vi "ntc_view.vi"() -> ()   [LabVIEW 2026]
uses:
  <vilib>/Instr/_visa.llb/VISA Configure Serial Port (Instr).vi
  <vilib>/express/express shared/transition.llb/Dynamic To Waveform Array.vi
  <vilib>/express/express signal manip/GetorSetDDTAttributes/Set DDT Attributes/SetT0.vi
  <vilib>/express/express shared/transition.llb/Waveform Array To Dynamic.vi
  <vilib>/express/express signal manip/GetorSetDDTAttributes/Set DDT Attributes/Set DDT Properties.xnode
panel:
  out "GOOD":bool
  out "Alarm <=  17 °C":bool
  out "Alarm\n >= 37 °C":bool caption="x >= y?"
  out "Linear Checker":cluster{"Tensão":dbl, "Waveform Chart":dbl}[](graph)
  out "Temperature Vs Time":dbl(graph)
  out "ADC Raw":u32
  out "Tensão":dbl(knob) scale=0.0..10.0
  out "Temperatura":dbl(slide) scale=17.0..37.0
  in  "stop":bool
  in  "VISA resource name":refnum<visa-resource-name>
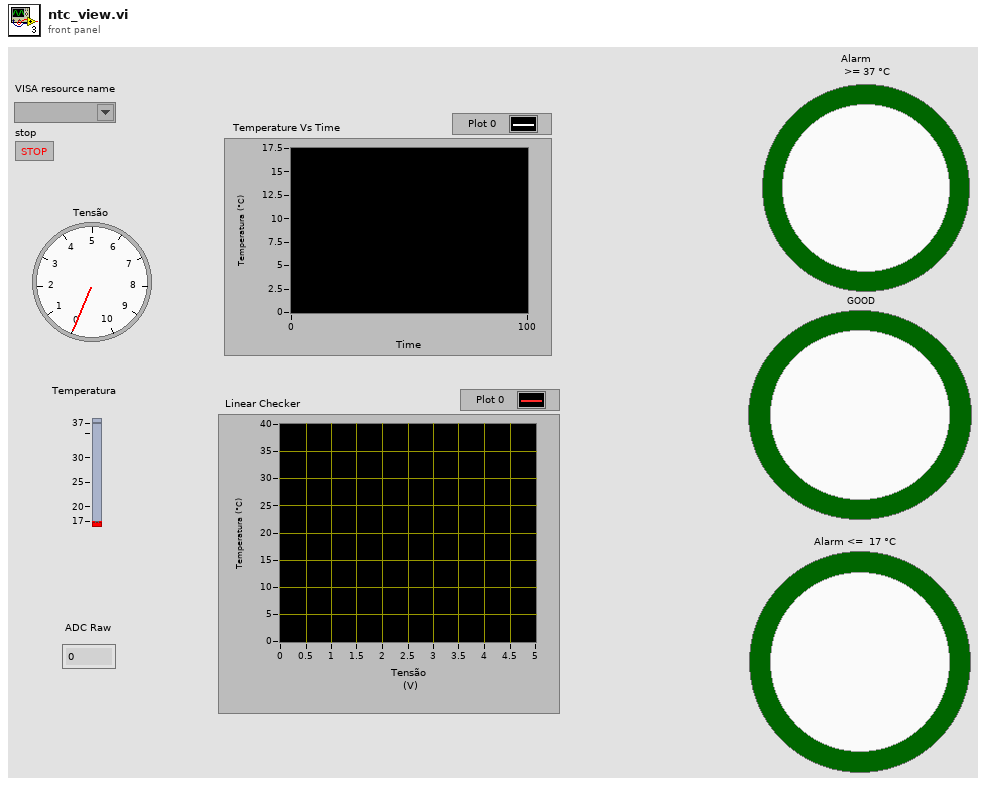
[diagram p1: front panel]
types:
  T1 = cluster{"Tensão":dbl, "Temperature Vs Time":dbl}[]
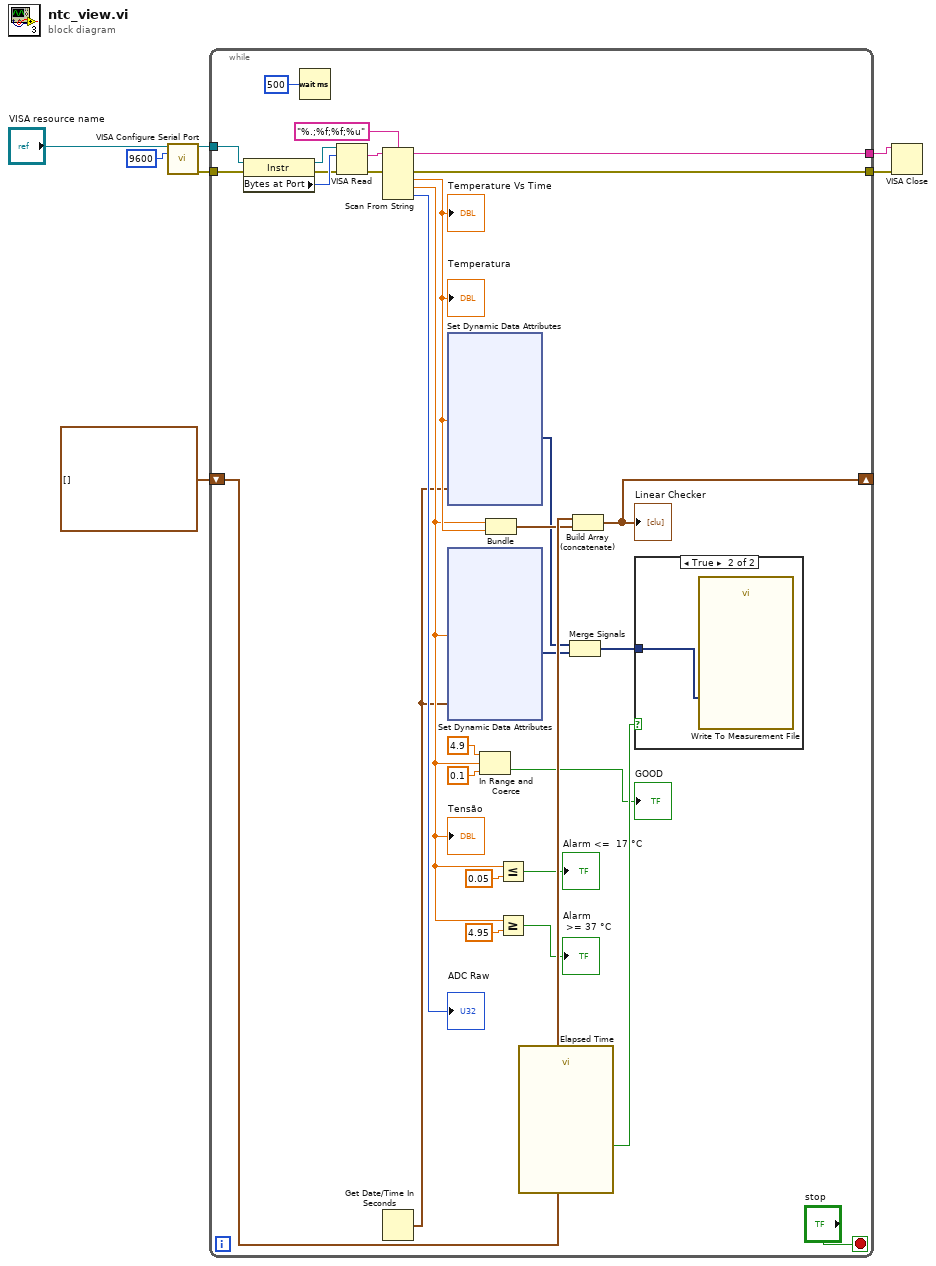
[diagram p0: block diagram]
diagram:
  n1 = call-poly "VISA Configure Serial Port"("VISA resource name"="VISA resource name", "baud rate (9600)"=u32 9600) -> ("VISA resource name out"=w6:refnum<visa-resource-name>, "error out"=w5:errorcluster)  [unwired: 12 in]
  n2 = while {
    tunnel: w6 -> [w32]
    tunnel: w5 -> [w33]
    tunnel: [w35] -> w4
    tunnel: [w34] -> w2
    shift-right: [w22] -> _
    shift-left: cluster{dbl, dbl}[] [] -> [w24]
    stop <- "stop" stop-if-true
    n3 = property class="Instr"(reference=w32, error in=w33) -> (reference out=w29:refnum<visa-resource-name>, error out=w28:errorcluster, "Bytes at Port"=w30:u32)
    n4 = Wait (ms)(milliseconds to wait=u32 500) -> ()  [unwired: 1 out]
    n5 = VISA Read(VISA resource name=w29, byte count=w30, error in (no error)=w28) -> (read buffer=w26:string, error out=w27:errorcluster)  [unwired: 2 out]
    n6 = Scan From String(format string="%.;%f;%f;%u", input string=w26, error in=w27) -> (remaining string=w34:string, error out=w35:errorcluster, output 1=w13:dbl, output 2=w12:dbl, output 3=→"ADC Raw":u32)  [unwired: 4 in, 1 out]
    "Temperatura" <- w13
    "Tensão" <- w12
    "Temperature Vs Time" <- w13
    n7 = Get Date/Time In Seconds() -> (seconds since 1Jan1904=w8:timestamp)
    n8 = xnode "Set Dynamic Data Attributes"("Signals In"=w13, "Timestamp"=w8) -> ("Signals Out"=w10:dynamicdata)  [unwired: 3 in, 1 out]
    n9 = xnode "Set Dynamic Data Attributes"("Signals In"=w12, "Timestamp"=w8) -> ("Signals Out"=w11:dynamicdata)  [unwired: 3 in, 1 out]
    n10 = In Range and Coerce(upper limit=4.9, x=w12, lower limit=0.1) -> (In Range?=→"GOOD":bool)  [unwired: 1 out]
    n11 = Bundle("Tensão"=w12, "Temperature Vs Time"=w13) -> (w23:cluster{"Tensão":dbl, "Temperature Vs Time":dbl})  [unwired: 1 in]
    n12 = Less Or Equal?(x=w12, y=0.05) -> (x <= y?=→"Alarm <=  17 °C":bool)
    n13 = Greater Or Equal?(x=w12, y=4.95) -> (x >= y?=→"Alarm\n >= 37 °C":bool)
    n14 = call "Elapsed Time"() -> ("Time has Elapsed"=w17:bool)  [unwired: 12 in, 7 out]
    n15 = Merge Signals(w10, w11) -> (w9:dynamicdata)
    n16 = Build Array (concatenate)(w24, w23) -> (w22:T1)
    "Linear Checker" <- w22
    n17 = case shown="True" w17 {
      tunnel: w9 -> [_ w74]
      frame False {
      }
      frame True {
        n18 = call "Write To Measurement File"("Signals"=w74) -> ()  [unwired: 16 in, 3 out]
      }
    }
  }
  n19 = VISA Close(VISA resource name=w2, error in (no error)=w4) -> ()  [unwired: 1 out]
